vi "Write Thermo Couple.vi"(10 "Thermo Couple":dbl, 11 "LabjacksController in":refnum<class "LabjacksController.lvclass">) -> (3 "LabjacksController out":refnum<class "LabjacksController.lvclass">)   [LabVIEW 2025, in "LabjacksController.lvclass"]
uses:
  LabjacksController.lvclass
  LabjacksController.lvclass/LabjacksController.ctl
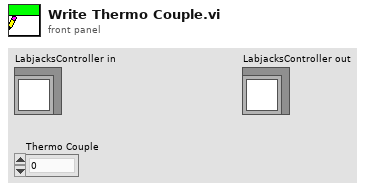
[diagram p1: front panel]
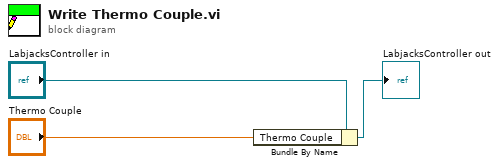
[diagram p0: block diagram]
diagram:
  n1 = Bundle By Name(cluster="LabjacksController in", "Thermo Couple"="Thermo Couple") -> (→"LabjacksController out":refnum<class "LabjacksController.lvclass">)
